vi "Test MQTT-6.0.0-3.vi"(8 "error in (no error)":errorcluster, 11 "Connection":refnum<class "Connection.lvclass">) -> (0 "error out":errorcluster, 3 "Connection":refnum<class "Connection.lvclass">)   [LabVIEW 2013]
uses:
  <vilib>/LabVIEW Open Source Project/Connection/Connection/Connection.lvclass
  <vilib>/LabVIEW Open Source Project/Connection/Connection.Websockets/Connection.WS.lvclass
  <vilib>/LabVIEW Open Source Project/Connection/Connection.Websockets/Connection.WS.lvclass/Connection.WS.ctl
  <vilib>/addons/_JKI Toolkits/Caraya/classes/Test/Test.lvclass
  <vilib>/addons/_JKI Toolkits/Caraya/classes/Assert/Assert.lvclass
panel:
  out "Value":string
  out "Supported Protocols":string[](array[string])
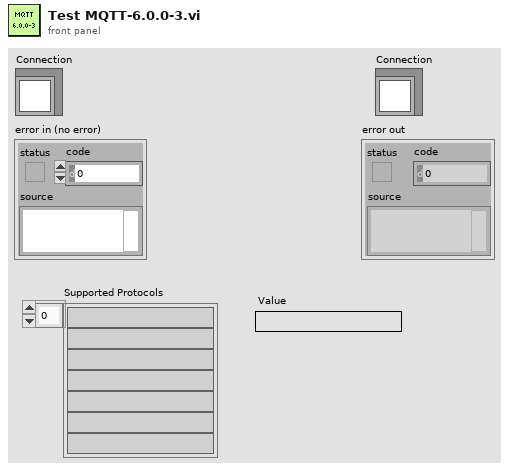
[diagram p1: front panel]
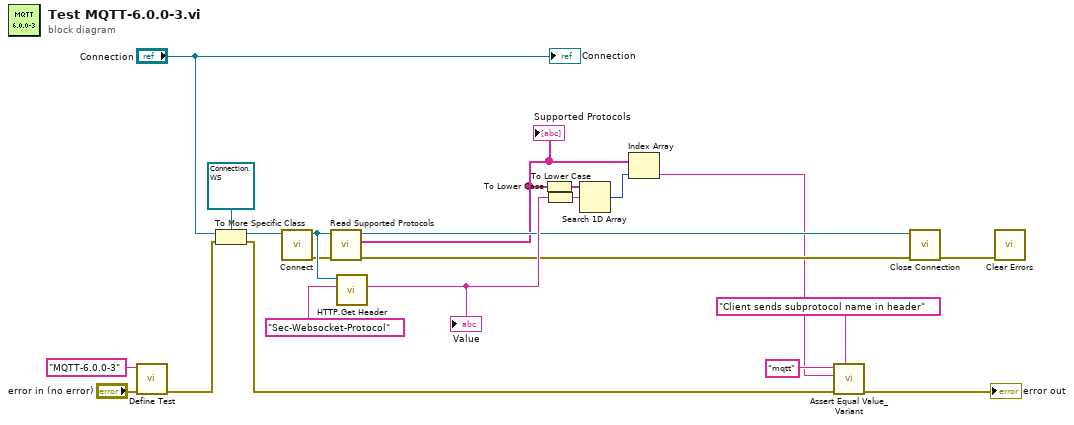
[diagram p0: block diagram]
diagram:
  n1 = call <vilib>:"Define Test.vi"("error in (no error)"="error in (no error)", "Label (VI Title)"="MQTT-6.0.0-3") -> ("error out"=w14:errorcluster)  [unwired: 9 in]
  n2 = To More Specific Class(target class=refnum<class "Connection.WS.lvclass"> refnum ("Connection.WS in"), reference="Connection", error in=w14) -> (specific class reference=w15:refnum<class "Connection.WS.lvclass">, error out=w13:errorcluster)
  n3 = call <vilib>:"Connect.vi"("Connection in"=w15) -> ("error out"=w5:errorcluster, "Connection out"=w7:refnum<class "Connection.WS.lvclass">)  [unwired: 9 in]
  n4 = call <vilib>:"Read Supported Protocols.vi"("error in (no error)"=w5, "Connection.WS in"=w7) -> ("error out"=w4:errorcluster, "Supported Protocols"=w3:string[], "Connection.WS out"=w6:refnum<class "Connection.WS.lvclass">)  [unwired: 6 in, 1 out]
  "Supported Protocols" <- w3
  n5 = call <vilib>:"HTTP.Get Header.vi"("Header Name"="Sec-Websocket-Protocol" ("name"), "Connection.WS in"=w7) -> ("Value"=w8:string)  [unwired: 6 in, 3 out]
  "Value" <- w8
  n6 = To Lower Case(string=w3) -> (all lower case string=w12:string[])
  n7 = To Lower Case(string=w8) -> (all lower case string=w11:string)
  n8 = Search 1D Array(1D array=w12, element=w11) -> (index of element=w10:i32)  [unwired: 1 in]
  n9 = Index Array(array=w3, index=w10) -> (element=w2:string)
  n10 = call <vilib>:"Assert Equal Value_Variant.vi"("Label"="Client sends subprotocol name in header", "error in (no error)"=w13, "Y"=w2, "X"="mqtt") -> ("error out"=→"error out":errorcluster)  [unwired: 7 in]
  n11 = call <vilib>:"Close Connection.vi"("error in (no error)"=w4, "Connection in"=w6) -> ("error out"=w17:errorcluster)  [unwired: 8 in, 1 out]
  n12 = call <vilib>:"Clear Errors.vi"("error in (no error)"=w17) -> ()  [unwired: 6 in, 1 out]
  "Connection" <- "Connection"
